vi "[ce] Is CE Engine DLL Loaded.vi"(8 "error in":errorcluster, 10 "system call (T)":bool=TRUE) -> (0 "error out":errorcluster, 2 "CE Engine DLL loaded":bool)   [LabVIEW 2021]
doc: "Returns TRUE if CalcExpress Engine DLL is currently loaded into memory.\n\n::: CalcExpress Toolkit :::\nCopyright (c) 2000-2026 Konstantin Shifershteyn. All rights reserved."
uses:
  kernel32.dll
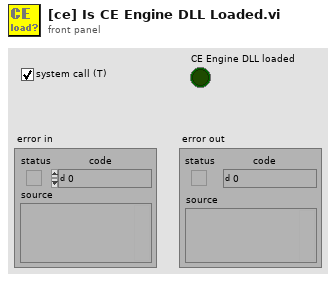
[diagram p1: front panel]
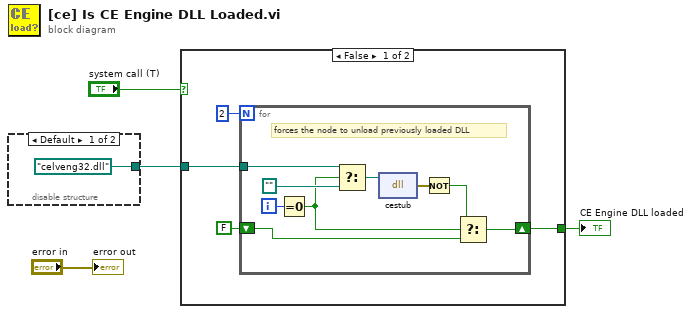
[diagram p0: block diagram]
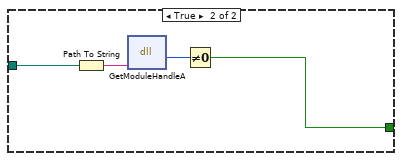
[diagram p2: hidden frame]
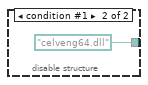
[diagram p3: hidden frame]
diagram:
  n1 = disable-structure shown="Default" {
    disable-tunnel: [path "celveng32.dll" path "celveng64.dll"] -> w2
    frame condition #0 (active) {
    }
    frame condition #1 {
    }
  }
  n2 = case shown="False" "system call (T)" {
    tunnel: [w8 w20] -> w4
    tunnel: w2 -> [w7 w21]
    frame False {
      n3 = for {
        N: 2 -> [_]
        shift-right: [w16] -> w8
        shift-left: FALSE -> [w13]
        tunnel: w7 -> [w12]
        i -> [w17]
        # "forces the node to unload previously loaded DLL"
        n4 = Equal To 0?(x=w17) -> (x = 0?=w14:bool)
        n5 = Select(t=w12, s=w14, f=path "") -> (s? t:f=w19:path)
        n6 = dll-call lib="C:/LV Projects/CalcExpress 26 LV85/vi.lib/addons/CalcExpress/cersrc/celveng.dll" fn="cestub" ("celveng.dll:msgAboutCE")(path in=w19) -> (error out=w11:errorcluster)  [unwired: 3 in, 1 out]
        n7 = Not(x=w11) -> (.not. x?=w15:bool)
        n8 = Select(t=w15, s=w14, f=w13) -> (s? t:f=w16:bool)
      }
    }
    frame True {
      n9 = Path To String(path=w21) -> (string=w22:string)
      n10 = dll-call lib="kernel32.dll" fn="GetModuleHandleA"("name"=w22) -> ("return type"=w23:u64)  [unwired: 4 in, 2 out]
      n11 = Not Equal To 0?(x=w23) -> (x != 0?=w20:bool)
    }
  }
  "CE Engine DLL loaded" <- w4
  "error out" <- "error in"
